vi "H3_Review_Me.vi"() -> ()   [LabVIEW 2018]
doc: "Use this template to build a VI to use as a subVI."
panel:
  in  "stop":bool
  in  "log file":path
  out "exactly 5 V":bool
  out "PASS":bool
  out "V":dbl
  in  "DMM":refnum<visa-resource-name>
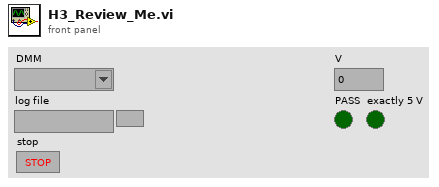
[diagram p1: front panel]
types:
  T1 = enum16{"open", "replace", "create", "open or create", "replace or create", "replace or create with confirmation"}
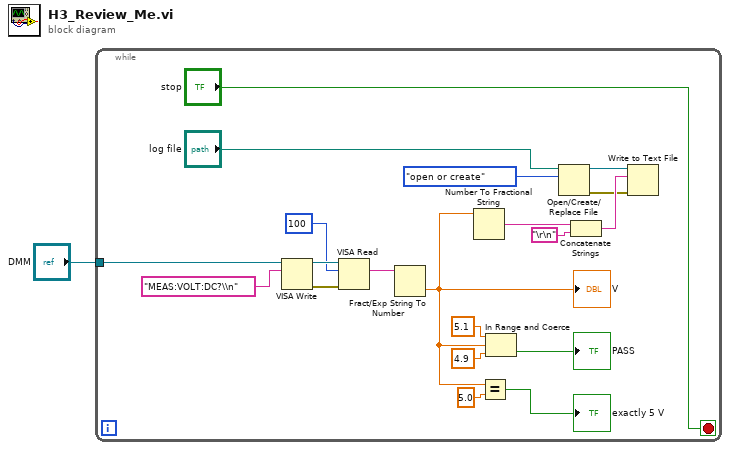
[diagram p0: block diagram]
diagram:
  n1 = while {
    tunnel: "DMM" -> [w21]
    stop <- "stop" stop-if-true
    n2 = VISA Write(VISA resource name=w21, write buffer="MEAS:VOLT:DC?\\n") -> (VISA resource name out=w19:refnum<visa-resource-name>, error out=w18:errorcluster)  [unwired: 1 in, 1 out]
    n3 = VISA Read(VISA resource name=w19, byte count=u32 100, error in (no error)=w18) -> (read buffer=w16:string)  [unwired: 3 out]
    n4 = Fract/Exp String To Number(string=w16) -> (number=w15:dbl)  [unwired: 3 in, 1 out]
    "V" <- w15
    n5 = Number To Fractional String(number=w15) -> (F-format string=w7:string)  [unwired: 3 in]
    n6 = Equal?(x=w15, y=5.0) -> (x = y?=→"exactly 5 V":bool)
    n7 = In Range and Coerce(upper limit=5.1, x=w15, lower limit=4.9) -> (In Range?=→"PASS":bool)  [unwired: 1 out]
    n8 = Open/Create/Replace File(file path (use dialog)="log file", operation (0:open)=T1."open or create") -> (refnum out=w5:refnum<file>, error out=w3:errorcluster)  [unwired: 4 in, 1 out]
    n9 = Concatenate Strings(w7, "\r\n" ("End of Line Constant")) -> (w4:string)
    n10 = Write to Text File(file (use dialog)=w5, text=w4, error in=w3) -> ()  [unwired: 1 in, 3 out]
  }
